vi "prop node.vi"() -> ()   [LabVIEW 2027]
uses:
  <vilib>/REVLibDriver/REVLibDriver.lvlib
  <resource>/objmgr/REVSpark.rc
panel:
  in  "IdleMode":u32(ring) items=["Coast", "Brake"]
  in  "stop":bool
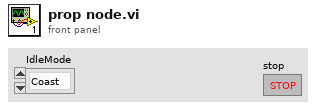
[diagram p1: front panel]
types:
  T1 = typedef "REVLibDriver.lvlib/REVSparkRefnum.ctl" = refnum<k20>
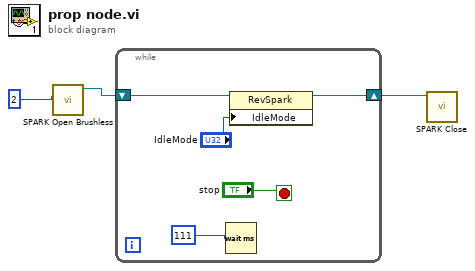
[diagram p0: block diagram]
diagram:
  n1 = call <vilib>:"SPARK Open Brushless.vi"("deviceId"=2) -> ("Spark refnum"=w3:T1)  [unwired: 9 in, 1 out]
  n2 = while {
    shift-right: [w7] -> w2
    shift-left: w3 -> [w8]
    stop <- "stop" stop-if-true
    n3 = Wait (ms)(milliseconds to wait=u32 111) -> ()  [unwired: 1 out]
    n4 = property class="RevSpark"(reference=w8, "IdleMode"="IdleMode") -> (reference out=w7:T1)  [unwired: 1 in, 1 out]
  }
  n5 = call <vilib>:"SPARK Close.vi"("Spark refnum"=w2) -> ()  [unwired: 10 in, 1 out]
